vi "Sum Of Doubles.vi"(0 "N":i32=3) -> (1 "Sum":i32, 2 "Count":i32)   [LabVIEW 2026]
doc: "Round21 nested-chain child (middle layer): a While Loop with two shift registers; each iteration calls Double It.vi on the iteration counter (iter+1) and accumulates the doubled value into Sum, so Sum = 2+4+...+2N = N*(N+1). Panel: N in (conIdx0, required), Sum out (conIdx1, recommended), Count out (conIdx2, recommended). Same loop dialect as the proven Accumulate N (R20): SR seeds stay on the root diagram, loop-internal constants enter via tunnels, stop condition is Greater Or Equal? feeding the Condition terminal. The Call sits INSIDE the loop; its terminal names are the callee's panel labels (x, Doubled) and its output net id (4253) is independent of the Call's uid (4252), per the round-6 recipe."
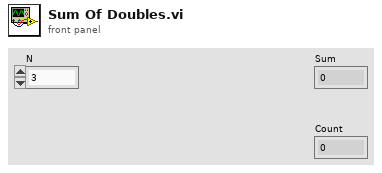
[diagram p1: front panel]
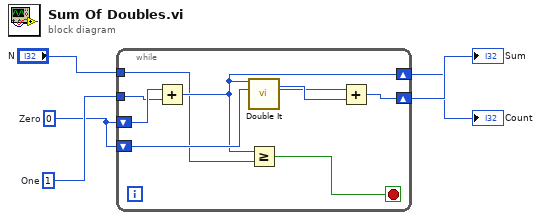
[diagram p0: block diagram]
diagram:
  w3 = 1  # One
  w2 = 0  # Zero
  n1 = while {
    tunnel: "N" -> [w6]
    tunnel: w3 -> [w7]
    shift-right: [w9] -> w4
    shift-left: w2 -> [w8]
    shift-right: [w11] -> w5
    shift-left: w2 -> [w10]
    stop <- w13 stop-if-true
    n2 = Add(x=w8, y=w7) -> (x+y=w9:i32)
    n3 = call "Double It.vi"("x"=w9) -> ("Doubled"=w12:i32)  [unwired: 14 in]
    n4 = Greater Or Equal?(x=w9, y=w6) -> (x >= y?=w13:bool)
    n5 = Add(x=w10, y=w12) -> (x+y=w11:i32)
  }
  "Sum" <- w5
  "Count" <- w4
